vi "PathPlanner_Path_CreatePath.vi"(11 "PathPlannerPath":T1={"Reversed"=FALSE, "RotationTargets"=[], "ConstraintZones"=[], "EventMarkers"=[], "GlobalConstraints"={"MaxVelocityMps;"=0.0, "MaxAccelerationMpsSq;"=0.0, "MaxAngularVelRadPsEc;"=0.0, "MaxAngularAccRadPSecSq"=0.0, "Exists"=FALSE, "Unlimited"=FALSE, "NominalVoltageVolts"=12.0}, "GoalEndState"={"VelocityMPS"=0.0, "Rotation"={"VALUE"=0.0, "COS"=1.0, "SIN"=0.0}}, "AllPoints"=[], "Name"="", "Waypoints"=[], "PointTowardsZones"=[], "IdealStartingState"={"VelocityMPS"=0.0, "Rotation"={"VALUE"=0.0, "COS"=1.0, "SIN"=0.0}}, "IsChoreoPath"=FALSE, "PreventFlipping"=FALSE} {"IdealStartingState"."Rotation"."SIN" format="%13.4f"; "IdealStartingState"."Rotation"."COS" format="%13.4f"; "IdealStartingState"."Rotation"."VALUE" format="%13.4f"; "PointTowardsZones"."TargetPosition"."Y" format="%14.3f"; "PointTowardsZones"."TargetPosition"."X" format="%14.3f"; "PointTowardsZones"."RotationOffset"."SIN" format="%13.4f"; "PointTowardsZones"."RotationOffset"."COS" format="%13.4f"; "PointTowardsZones"."RotationOffset"."VALUE" format="%13.4f"; "Waypoints"."nextControl"."Y" format="%14.3f"; "Waypoints"."nextControl"."X" format="%14.3f"; "Waypoints"."anchor"."Y" format="%14.3f"; "Waypoints"."anchor"."X" format="%14.3f"; "Waypoints"."prevControl"."Y" format="%14.3f"; "Waypoints"."prevControl"."X" format="%14.3f"; "AllPoints"."RotationTarget"."rotation"."SIN" format="%13.4f"; "AllPoints"."RotationTarget"."rotation"."COS" format="%13.4f"; "AllPoints"."RotationTarget"."rotation"."VALUE" format="%13.4f"; "AllPoints"."Position"."Y" format="%14.3f"; "AllPoints"."Position"."X" format="%14.3f"; "GoalEndState"."Rotation"."SIN" format="%13.4f"; "GoalEndState"."Rotation"."COS" format="%13.4f"; "GoalEndState"."Rotation"."VALUE" format="%13.4f"; "RotationTargets"."rotation"."SIN" format="%13.4f"; "RotationTargets"."rotation"."COS" format="%13.4f"; "RotationTargets"."rotation"."VALUE" format="%13.4f"}) -> (0 "Error":bool, 3 "Points":T11[](array[typedef]) {"RotationTarget"."rotation"."SIN" format="%13.4f"; "RotationTarget"."rotation"."COS" format="%13.4f"; "RotationTarget"."rotation"."VALUE" format="%13.4f"; "Position"."Y" format="%14.3f"; "Position"."X" format="%14.3f"})   [LabVIEW 2019, in "PathPlanner24.lvlib"]
doc: "Create the path points for this path. This is an internal function.\n\nInputs: \n - PathPlannerPath - cluster - Path definition data structure\n\nOutputs:\n - PathPoints - PathPoint array - Array of points along the path\n - Error - boolean - TRUE if an error occured."
uses:
  PathPlanner24.lvlib
  <vilib>/Rock Robotics/WPI/ThirdParty/JAS_Junk/TrajLib/TypeDef/TRANSLATION2D.ctl
  <vilib>/Rock Robotics/WPI/ThirdParty/JAS_Junk/TrajLib/Trajectory_Library.lvlib
  <vilib>/Rock Robotics/WPI/ThirdParty/JAS_Junk/TrajLib/TypeDef/ROTATION2D.ctl
  TypeDef/PathPlannerPathConstraints.ctl
  TypeDef/PathPlannerPathPoint.ctl
  TypeDef/PathPlannerRotationTarget.ctl
  TypeDef/PathPlannerConstraintsZone.ctl
  ENum/PathPlanner_TrajectoryEvent_Type_ENUM.ctl
  TypeDef/PathPlannerCommandUtil.ctl
  TypeDef/PathPlannerEventMarker.ctl
  TypeDef/PathPlannerGoalEndState.ctl
  TypeDef/PathPlannerWaypoint.ctl
  TypeDef/PathPlannerPointTowardsZone.ctl
  TypeDef/PathPlannerIdealStartingState.ctl
  TypeDef/PathPlannerPath.ctl
  ENum/PathPlanner_CommandUtil_Type_ENUM.ctl
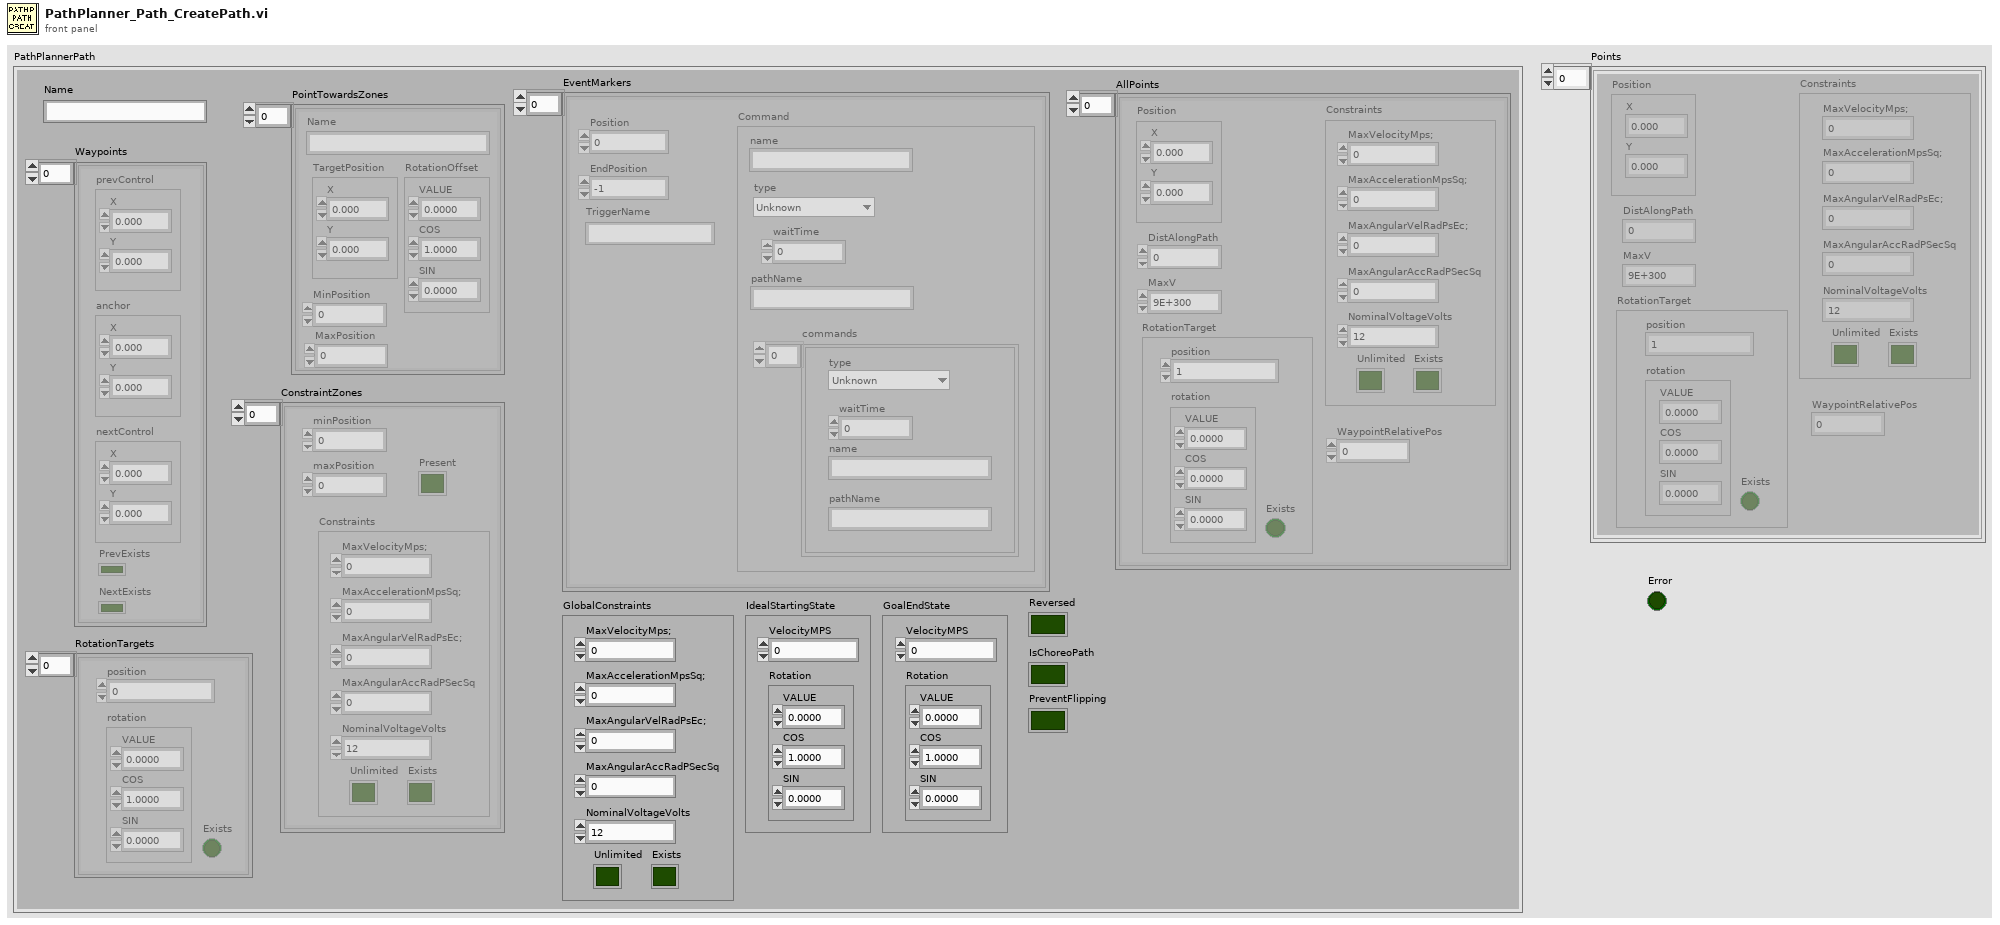
[diagram p1: front panel]
types:
  T1 = typedef "PathPlanner24.lvlib/PathPlannerPath.ctl" = cluster{"Reversed":bool, "RotationTargets":T2[], "ConstraintZones":T4[], "EventMarkers":T6[], "GlobalConstraints":T5, "GoalEndState":T10, "AllPoints":T11[], "Name":string, "Waypoints":T13[], "PointTowardsZones":T14[], "IdealStartingState":T15, "IsChoreoPath":bool, "PreventFlipping":bool}
  T2 = typedef "PathPlanner24.lvlib/PathPlannerRotationTarget.ctl" = cluster{"position":dbl, "rotation":T3, "Exists":bool}
  T3 = typedef "Trajectory_Library.lvlib/ROTATION2D.ctl" = cluster{"VALUE":dbl, "COS":dbl, "SIN":dbl}
  T4 = typedef "PathPlanner24.lvlib/PathPlannerConstraintsZone.ctl" = cluster{"minPosition":dbl, "maxPosition":dbl, "Constraints":T5, "Present":bool}
  T5 = typedef "PathPlanner24.lvlib/PathPlannerPathConstraints.ctl" = cluster{"MaxVelocityMps;":dbl, "MaxAccelerationMpsSq;":dbl, "MaxAngularVelRadPsEc;":dbl, "MaxAngularAccRadPSecSq":dbl, "Exists":bool, "Unlimited":bool, "NominalVoltageVolts":dbl}
  T6 = typedef "PathPlanner24.lvlib/PathPlannerEventMarker.ctl" = cluster{"Position":dbl, "Command":T7, "TriggerName":string, "EndPosition":dbl}
  T7 = typedef "PathPlanner24.lvlib/PathPlannerCommandUtil.ctl" = cluster{"waitTime":dbl, "name":string, "pathName":string, "commands":cluster{"type":T8, "waitTime":dbl, "name":string, "pathName":string}[], "type":T9}
  T8 = typedef "PathPlanner24.lvlib/PathPlanner_TrajectoryEvent_Type_ENUM.ctl" = enum16{"Unknown", "Wait", "Named", "Path", "Sequential", "Parallel", "Race", "Deadline", "PointTowardsZoneEnter", "PointTowardsZoneExit", "TriggerEventStart", "TriggerEventStop", "TriggerEventOneshot"}
  T9 = typedef "PathPlanner24.lvlib/PathPlanner_CommandUtil_Type_ENUM.ctl" = enum16{"Unknown", "Wait", "Named", "Path", "Sequential", "Parallel", "Race", "Deadline"}
  T10 = typedef "PathPlanner24.lvlib/PathPlannerGoalEndState.ctl" = cluster{"VelocityMPS":dbl, "Rotation":T3}
  T11 = typedef "PathPlanner24.lvlib/PathPlannerPathPoint.ctl" = cluster{"Position":T12, "DistAlongPath":dbl, "MaxV":dbl, "Constraints":T5, "RotationTarget":T2, "WaypointRelativePos":dbl}
  T12 = typedef "Trajectory_Library.lvlib/TRANSLATION2D.ctl" = cluster{"X":dbl, "Y":dbl}
  T13 = typedef "PathPlanner24.lvlib/PathPlannerWaypoint.ctl" = cluster{"prevControl":T12, "anchor":T12, "nextControl":T12, "PrevExists":bool, "NextExists":bool}
  T14 = typedef "PathPlanner24.lvlib/PathPlannerPointTowardsZone.ctl" = cluster{"RotationOffset":T3, "Name":string, "TargetPosition":T12, "MinPosition":dbl, "MaxPosition":dbl}
  T15 = typedef "PathPlanner24.lvlib/PathPlannerIdealStartingState.ctl" = cluster{"VelocityMPS":dbl, "Rotation":T3}
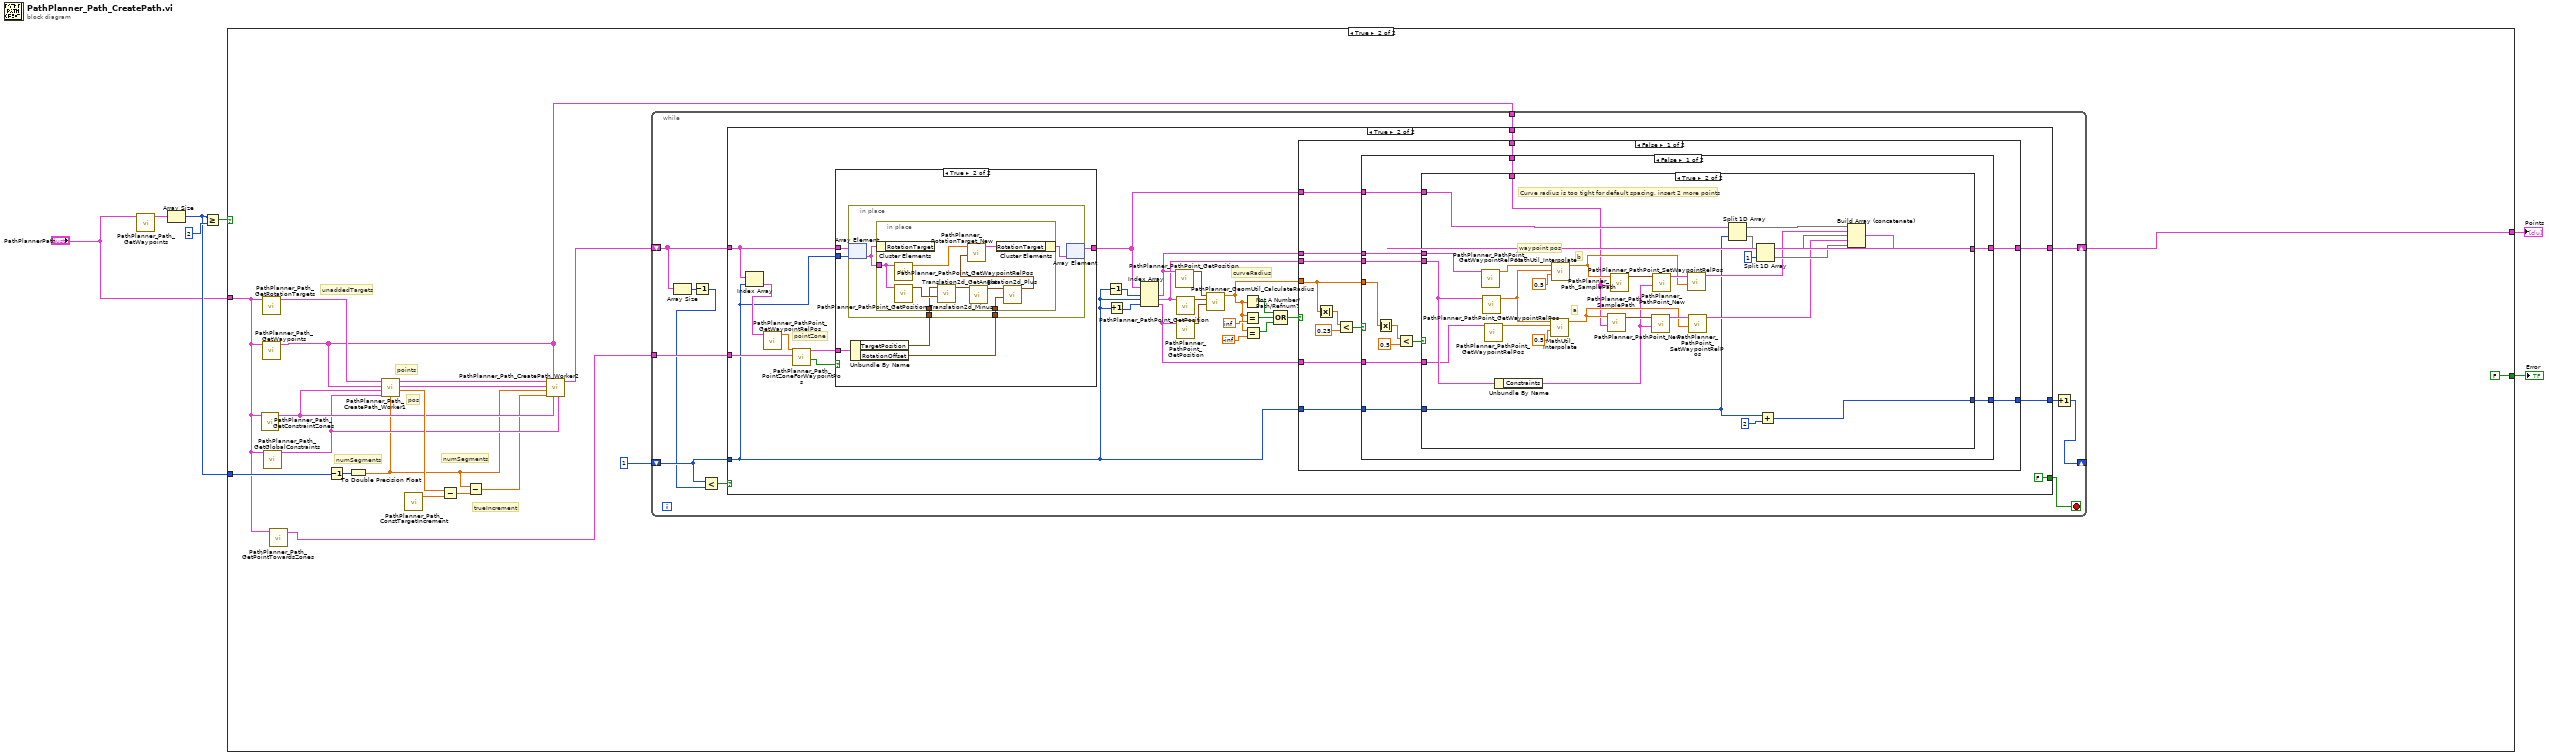
[diagram p0: block diagram]
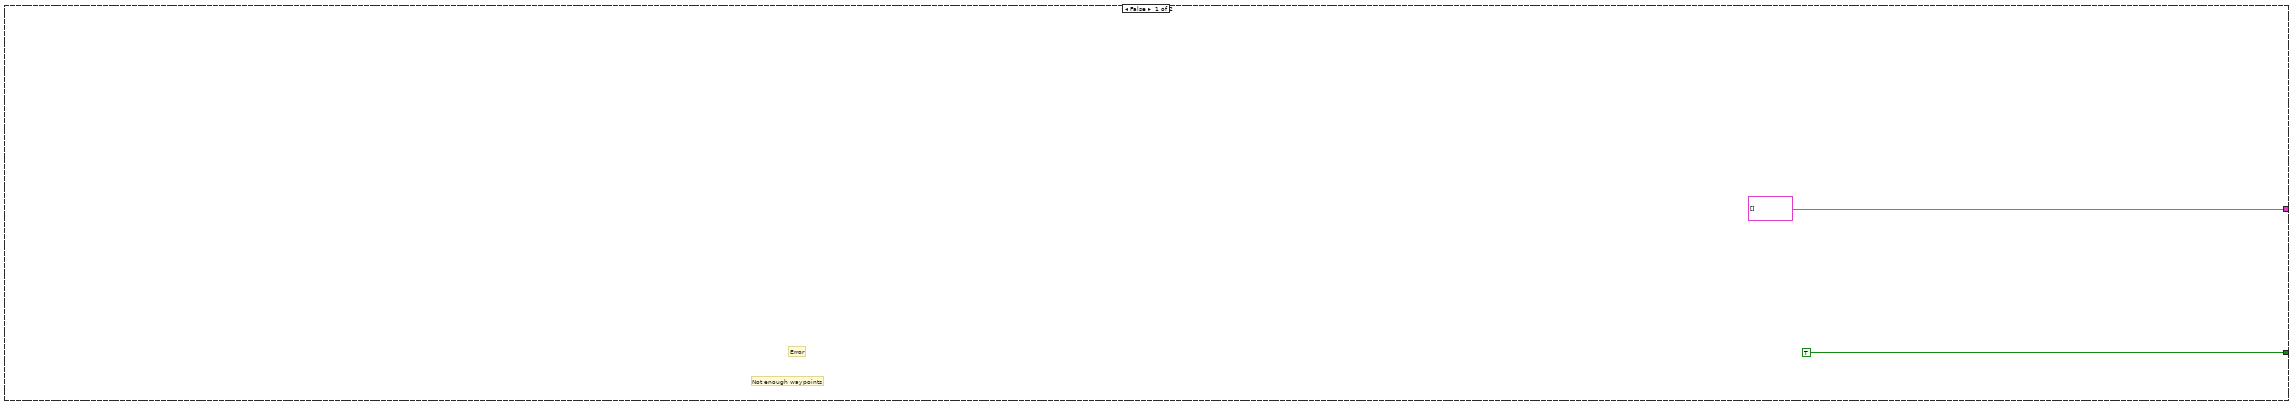
[diagram p2: hidden frame]
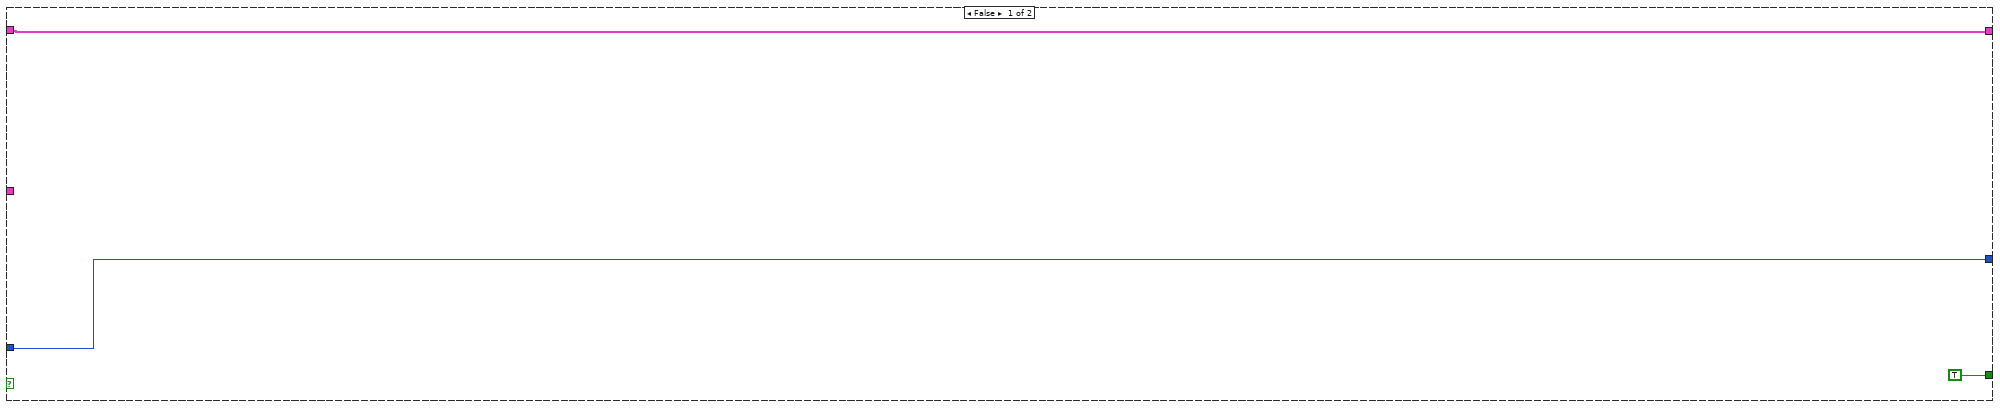
[diagram p3: hidden frame]
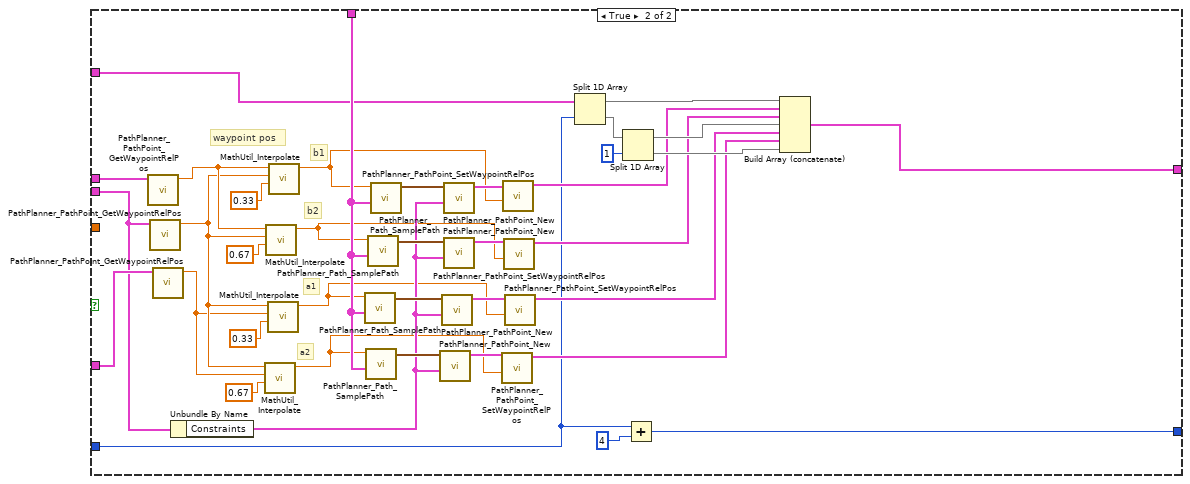
[diagram p5: hidden frame]
diagram:
  n1 = call "PathPlanner_Path_GetWaypoints.vi"("PathPlannerPath"="PathPlannerPath") -> ("Waypoints"=w2:T13[])  [unwired: 10 in]
  n2 = Array Size(array=w2) -> (size(s)=w3:i32)
  n3 = Greater Or Equal?(x=w3, y=2) -> (x >= y?=w6:bool)
  n4 = case shown="True" w6 {
    tunnel: [TRUE FALSE] -> w5
    tunnel: [T11[] [] ("Points") w14] -> w4
    tunnel: w3 -> [_ w27]
    tunnel: "PathPlannerPath" -> [_ w16]
    frame False {
      # "Not enough waypoints"
      # "Error"
    }
    frame True {
      # "numSegments"
      # "trueIncrement"
      # "pos"
      # "points"
      # "numSegments"
      # "unaddedTargets"
      n5 = call "PathPlanner_Path_GetConstraintZones.vi"("PathPlannerPath"=w16) -> ("ConstraintZones"=w20:T4[])  [unwired: 10 in]
      n6 = call "PathPlanner_Path_GetRotationTargets.vi"("PathPlannerPath"=w16) -> ("RotationTargets"=w25:T2[])  [unwired: 10 in]
      n7 = call "PathPlanner_Path_GetWaypoints.vi"("PathPlannerPath"=w16) -> ("Waypoints"=w13:T13[])  [unwired: 10 in]
      n8 = call "PathPlanner_Path_GetGlobalConstraints.vi"("PathPlannerPath"=w16) -> ("GlobalConstraints"=w19:T5)  [unwired: 10 in]
      n9 = call "PathPlanner_Path_GetPointTowardsZones.vi"("PathPlannerPath"=w16) -> ("PointTowardsZones"=w15:T14[])  [unwired: 10 in]
      n10 = Decrement(x=w27) -> (x-1=w26:i32)
      n11 = To Double Precision Float(number=w26) -> (double precision float=w18:dbl)
      n12 = call "PathPlanner_Path_CreatePath_Worker1.vi"("LargestWaypointIndex"=w18, "GlobalConstraints"=w19, "ConstraintZones"=w20, "Waypoints"=w13, "RotationTargets"=w25) -> ("pos"=w24:dbl, "UnaddedTargets"=w21:T2[], "Points"=w11:T11[])  [unwired: 4 in]
      n13 = call "PathPlanner_Path_ConstTargetIncrement.vi"() -> ("TargetIncrement"=w23:dbl)  [unwired: 11 in]
      n14 = Subtract(x=w24, y=w23) -> (x-y=w22:dbl)
      n15 = Subtract(x=w18, y=w22) -> (x-y=w17:dbl)
      n16 = call "PathPlanner_Path_CreatePath_Worker2.vi"("GlobalConstraints"=w19, "ConstraintZones"=w20, "Waypoints"=w13, "TrueIncrement"=w17, "NumSegments"=w18, "UnaddedTargets"=w21, "Points in"=w11) -> ("Points out"=w10:T11[])  [unwired: 4 in]
      n17 = while {
        tunnel: w15 -> [w39]
        shift-right: [w38] -> w14
        shift-left: w10 -> [w34]
        tunnel: w13 -> [w37]
        shift-right: [w29] -> _
        shift-left: 1 -> [w36]
        stop <- w31 stop-if-true
        n18 = Array Size(array=w34) -> (size(s)=w35:i32)
        n19 = Decrement(x=w35) -> (x-1=w32:i32)
        n20 = Less?(x=w36, y=w32) -> (x < y?=w33:bool)
        n21 = case shown="True" w33 {
          tunnel: w36 -> [w40 w43]
          tunnel: w39 -> [_ w69]
          tunnel: w34 -> [w42 w65]
          tunnel: [w42 w51] -> w38
          tunnel: w37 -> [_ w46]
          tunnel: [TRUE FALSE] -> w31
          tunnel: [w40 w44] -> w30
          frame False {
          }
          frame True {
            # "curveRadius"
            # "pointZone"
            n22 = Index Array(array=w65, index=w43) -> (element=w64:T11)
            n23 = call "PathPlanner_PathPoint_GetWaypointRelPos.vi"("PathPlannerPoint"=w64) -> ("WaypointRelativePos"=w68:dbl)  [unwired: 10 in]
            n24 = call "PathPlanner_Path_PointZoneForWaypointPos.vi"("PointTowardsZone"=w69, "Pos"=w68) -> ("Found"=w67:bool, "outPointTowardsZone"=w66:T14)  [unwired: 8 in]
            n25 = case shown="True" w67 {
              tunnel: w65 -> [w164 w169]
              tunnel: w66 -> [_ w170]
              tunnel: w43 -> [_ w168]
              tunnel: [w164 w167] -> w52
              frame False {
              }
              frame True {
                n26 = Unbundle By Name(w170) -> ("TargetPosition"=w166:T12, "RotationOffset"=w165:T3)
                n27 = in-place {
                  in-place-border: w166 -> [w172]
                  in-place-border: w165 -> [w171]
                  n28 = in-place-array #1(w169, w168) -> (w174:T11)
                  n29 = in-place {
                    in-place-border: w174 -> [w181]
                    in-place-border: w172 -> [w179]
                    in-place-border: w171 -> [w177]
                    n30 = in-place-cluster #2(w174) -> ()  [unwired: 1 out]
                    n31 = call "PathPlanner_PathPoint_GetPosition.vi"("PathPlannerPoint"=w181) -> ("Position"=w180:T12)  [unwired: 10 in]
                    n32 = call "PathPlanner_PathPoint_GetWaypointRelPos.vi"("PathPlannerPoint"=w181) -> ("WaypointRelativePos"=w182:dbl)  [unwired: 10 in]
                    n33 = call <vilib>:"Translation2d_Minus.vi"("other Translation"=w180, "In Translation"=w179) -> ("Out Translation"=w178:T12)  [unwired: 9 in]
                    n34 = call <vilib>:"Translation2d_GetAngle.vi"("In Translation"=w178) -> ("Angle_Rotation2d"=w176:T3)  [unwired: 10 in]
                    n35 = call <vilib>:"Rotation2d_Plus.vi"("other ROTATION"=w177, "in ROTATION"=w176) -> ("out ROTATION"=w175:T3)  [unwired: 9 in]
                    n36 = call "PathPlanner_RotationTarget_New.vi"("rotation"=w175, "position"=w182) -> ("RotationTarget"=w183:T2)  [unwired: 9 in]
                    n37 = in-place-cluster #2("RotationTarget"=w183) -> (w173:T11)
                  }
                  n38 = in-place-array #1(w173) -> (w167:T11[])  [unwired: 1 out]
                }
              }
            }
            n39 = Decrement(x=w43) -> (x-1=w63:i32)
            n40 = Increment(x=w43) -> (x+1=w62:i32)
            n41 = Index Array(array=w52, index #1=w63, index #2=w43, index #3=w62) -> (element #1=w49:T11, element #2=w48:T11, element #3=w47:T11)
            n42 = call "PathPlanner_PathPoint_GetPosition.vi"("PathPlannerPoint"=w49) -> ("Position"=w61:T12)  [unwired: 10 in]
            n43 = call "PathPlanner_PathPoint_GetPosition.vi"("PathPlannerPoint"=w48) -> ("Position"=w60:T12)  [unwired: 10 in]
            n44 = call "PathPlanner_PathPoint_GetPosition.vi"("PathPlannerPoint"=w47) -> ("Position"=w59:T12)  [unwired: 10 in]
            n45 = call "PathPlanner_GeomUtil_CalculateRadius.vi"("C"=w59, "B"=w60, "A"=w61) -> ("Radius"=w50:dbl)  [unwired: 8 in]
            n46 = Not A Number/Path/Refnum?(number/path/refnum=w50) -> (NaN/Path/Refnum?=w58:bool)
            n47 = Equal?(x=w50, y=inf) -> (x = y?=w57:bool)
            n48 = Equal?(x=w50, y=-inf) -> (x = y?=w56:bool)
            n49 = Compound Arithmetic op=OR(w58, w57, w56) -> (w53:bool)
            n50 = case shown="False" w53 {
              tunnel: w52 -> [w74 w163]
              tunnel: [w73 w163] -> w51
              tunnel: w50 -> [w70 _]
              tunnel: w49 -> [w78 _]
              tunnel: w48 -> [w77 _]
              tunnel: w47 -> [w76 _]
              tunnel: w46 -> [w75 _]
              tunnel: [w72 w162] -> w44
              tunnel: w43 -> [w71 w162]
              frame False {
                n51 = Absolute Value(x=w70) -> (abs(x)=w80:dbl)
                n52 = Less?(x=w80, y=0.25) -> (x < y?=w79:bool)
                n53 = case shown="False" w79 {
                  tunnel: w78 -> [w85 w161]
                  tunnel: w77 -> [w84 w152]
                  tunnel: w76 -> [w83 w160]
                  tunnel: w75 -> [w82 w147]
                  tunnel: w74 -> [w90 w145]
                  tunnel: [w89 w127] -> w73
                  tunnel: [w87 w125] -> w72
                  tunnel: w71 -> [w88 w124]
                  tunnel: w70 -> [w91 _]
                  frame False {
                    n54 = Absolute Value(x=w91) -> (abs(x)=w92:dbl)
                    n55 = Less?(x=w92, y=0.5) -> (x < y?=w86:bool)
                    n56 = case shown="True" w86 {
                      tunnel: w90 -> [w95 w104]
                      tunnel: [w95 w96] -> w89
                      tunnel: w88 -> [w94 w98]
                      tunnel: [w94 w97] -> w87
                      tunnel: w85 -> [_ w103]
                      tunnel: w84 -> [_ w102]
                      tunnel: w83 -> [_ w101]
                      tunnel: w82 -> [_ w100]
                      frame False {
                      }
                      frame True {
                        # "a"
                        # "b"
                        # "waypoint pos"
                        # "Curve radius is too tight for default spacing, insert 2 more points"
                        n57 = call "PathPlanner_PathPoint_GetWaypointRelPos.vi"("PathPlannerPoint"=w103) -> ("WaypointRelativePos"=w122:dbl)  [unwired: 10 in]
                        n58 = call "PathPlanner_PathPoint_GetWaypointRelPos.vi"("PathPlannerPoint"=w102) -> ("WaypointRelativePos"=w120:dbl)  [unwired: 10 in]
                        n59 = call "PathPlanner_PathPoint_GetWaypointRelPos.vi"("PathPlannerPoint"=w101) -> ("WaypointRelativePos"=w119:dbl)  [unwired: 10 in]
                        n60 = Unbundle By Name(w102) -> ("Constraints"=w99:T5)
                        n61 = call <vilib>:"MathUtil_Interpolate.vi"("T"=0.5, "EndValue"=w119, "StartValue"=w120) -> ("InterpolatedValue"=w106:dbl)  [unwired: 8 in]
                        n62 = call <vilib>:"MathUtil_Interpolate.vi"("T"=0.5, "EndValue"=w120, "StartValue"=w122) -> ("InterpolatedValue"=w107:dbl)  [unwired: 8 in]
                        n63 = call "PathPlanner_Path_SamplePath.vi"("Waypoints"=w100, "WaypointRelativePos"=w106) -> ("Sample"=w117:T12)  [unwired: 9 in]
                        n64 = call "PathPlanner_Path_SamplePath.vi"("Waypoints"=w100, "WaypointRelativePos"=w107) -> ("Sample"=w118:T12)  [unwired: 9 in]
                        n65 = call "PathPlanner_PathPoint_New.vi"("Constraints"=w99, "Position"=w117) -> ("PathPlannerPoint"=w110:T11)  [unwired: 9 in]
                        n66 = call "PathPlanner_PathPoint_New.vi"("Constraints"=w99, "Position"=w118) -> ("PathPlannerPoint"=w111:T11)  [unwired: 9 in]
                        n67 = call "PathPlanner_PathPoint_SetWaypointRelPos.vi"("WaypointRelativePos"=w107, "PathPlannerPoint"=w111) -> ("outPathPlannerPoint"=w109:T11)  [unwired: 9 in]
                        n68 = call "PathPlanner_PathPoint_SetWaypointRelPos.vi"("WaypointRelativePos"=w106, "PathPlannerPoint"=w110) -> ("outPathPlannerPoint"=w108:T11)  [unwired: 9 in]
                        n69 = Split 1D Array(array=w104, index=w98) -> (first subarray=w116:T11[], second subarray=w115:T11[])
                        n70 = Split 1D Array(array=w115, index=1) -> (first subarray=w113:T11[], second subarray=w112:T11[])
                        n71 = Add(x=w98, y=2) -> (x+y=w97:i32)
                        n72 = Build Array (concatenate)(w116, w109, w113, w108, w112) -> (w96:T11[])
                      }
                    }
                  }
                  frame True {
                    # "a2"
                    # "a1"
                    # "b2"
                    # "b1"
                    # "waypoint pos"
                    n73 = call "PathPlanner_PathPoint_GetWaypointRelPos.vi"("PathPlannerPoint"=w161) -> ("WaypointRelativePos"=w157:dbl)  [unwired: 10 in]
                    n74 = call "PathPlanner_PathPoint_GetWaypointRelPos.vi"("PathPlannerPoint"=w152) -> ("WaypointRelativePos"=w154:dbl)  [unwired: 10 in]
                    n75 = call "PathPlanner_PathPoint_GetWaypointRelPos.vi"("PathPlannerPoint"=w160) -> ("WaypointRelativePos"=w153:dbl)  [unwired: 10 in]
                    n76 = Unbundle By Name(w152) -> ("Constraints"=w146:T5)
                    n77 = call <vilib>:"MathUtil_Interpolate.vi"("T"=0.67, "EndValue"=w153, "StartValue"=w154) -> ("InterpolatedValue"=w128:dbl)  [unwired: 8 in]
                    n78 = call <vilib>:"MathUtil_Interpolate.vi"("T"=0.67, "EndValue"=w154, "StartValue"=w157) -> ("InterpolatedValue"=w130:dbl)  [unwired: 8 in]
                    n79 = call <vilib>:"MathUtil_Interpolate.vi"("T"=0.33, "EndValue"=w153, "StartValue"=w154) -> ("InterpolatedValue"=w129:dbl)  [unwired: 8 in]
                    n80 = call <vilib>:"MathUtil_Interpolate.vi"("T"=0.33, "EndValue"=w154, "StartValue"=w157) -> ("InterpolatedValue"=w131:dbl)  [unwired: 8 in]
                    n81 = call "PathPlanner_Path_SamplePath.vi"("Waypoints"=w147, "WaypointRelativePos"=w129) -> ("Sample"=w149:T12)  [unwired: 9 in]
                    n82 = call "PathPlanner_Path_SamplePath.vi"("Waypoints"=w147, "WaypointRelativePos"=w128) -> ("Sample"=w148:T12)  [unwired: 9 in]
                    n83 = call "PathPlanner_Path_SamplePath.vi"("Waypoints"=w147, "WaypointRelativePos"=w130) -> ("Sample"=w150:T12)  [unwired: 9 in]
                    n84 = call "PathPlanner_Path_SamplePath.vi"("Waypoints"=w147, "WaypointRelativePos"=w131) -> ("Sample"=w151:T12)  [unwired: 9 in]
                    n85 = call "PathPlanner_PathPoint_New.vi"("Constraints"=w146, "Position"=w148) -> ("PathPlannerPoint"=w136:T11)  [unwired: 9 in]
                    n86 = call "PathPlanner_PathPoint_New.vi"("Constraints"=w146, "Position"=w149) -> ("PathPlannerPoint"=w137:T11)  [unwired: 9 in]
                    n87 = call "PathPlanner_PathPoint_New.vi"("Constraints"=w146, "Position"=w151) -> ("PathPlannerPoint"=w139:T11)  [unwired: 9 in]
                    n88 = call "PathPlanner_PathPoint_New.vi"("Constraints"=w146, "Position"=w150) -> ("PathPlannerPoint"=w138:T11)  [unwired: 9 in]
                    n89 = call "PathPlanner_PathPoint_SetWaypointRelPos.vi"("WaypointRelativePos"=w128, "PathPlannerPoint"=w136) -> ("outPathPlannerPoint"=w132:T11)  [unwired: 9 in]
                    n90 = call "PathPlanner_PathPoint_SetWaypointRelPos.vi"("WaypointRelativePos"=w131, "PathPlannerPoint"=w139) -> ("outPathPlannerPoint"=w135:T11)  [unwired: 9 in]
                    n91 = call "PathPlanner_PathPoint_SetWaypointRelPos.vi"("WaypointRelativePos"=w130, "PathPlannerPoint"=w138) -> ("outPathPlannerPoint"=w134:T11)  [unwired: 9 in]
                    n92 = call "PathPlanner_PathPoint_SetWaypointRelPos.vi"("WaypointRelativePos"=w129, "PathPlannerPoint"=w137) -> ("outPathPlannerPoint"=w133:T11)  [unwired: 9 in]
                    n93 = Split 1D Array(array=w145, index=w124) -> (first subarray=w144:T11[], second subarray=w143:T11[])
                    n94 = Split 1D Array(array=w143, index=1) -> (first subarray=w141:T11[], second subarray=w140:T11[])
                    n95 = Add(x=w124, y=4) -> (x+y=w125:i32)
                    n96 = Build Array (concatenate)(w144, w135, w134, w141, w133, w132, w140) -> (w127:T11[])
                  }
                }
              }
              frame True {
                # "bad radius number"
              }
            }
          }
        }
        n97 = Increment(x=w30) -> (x+1=w29:i32)
      }
    }
  }
  "Error" <- w5
  "Points" <- w4
